vi "Motion_one_way_ver2_lin_sin.vi"(7 "Parameters":T1={"T"=2000.0, "Linear or sine?"=0.0, "Buffer size"=0.5, "Buffer power"=3.0}, 8 "Error IN":errorcluster, 9 "previousSTATE":dbl[][](array[numeric]), 10 "nextSTATE":dbl[][](array[numeric]), 11 "Constants IN":T3) -> (0 "Error OUT":errorcluster, 2 "Motion Sequence":T2, 3 "Constants OUT":T3)   [LabVIEW 2019]
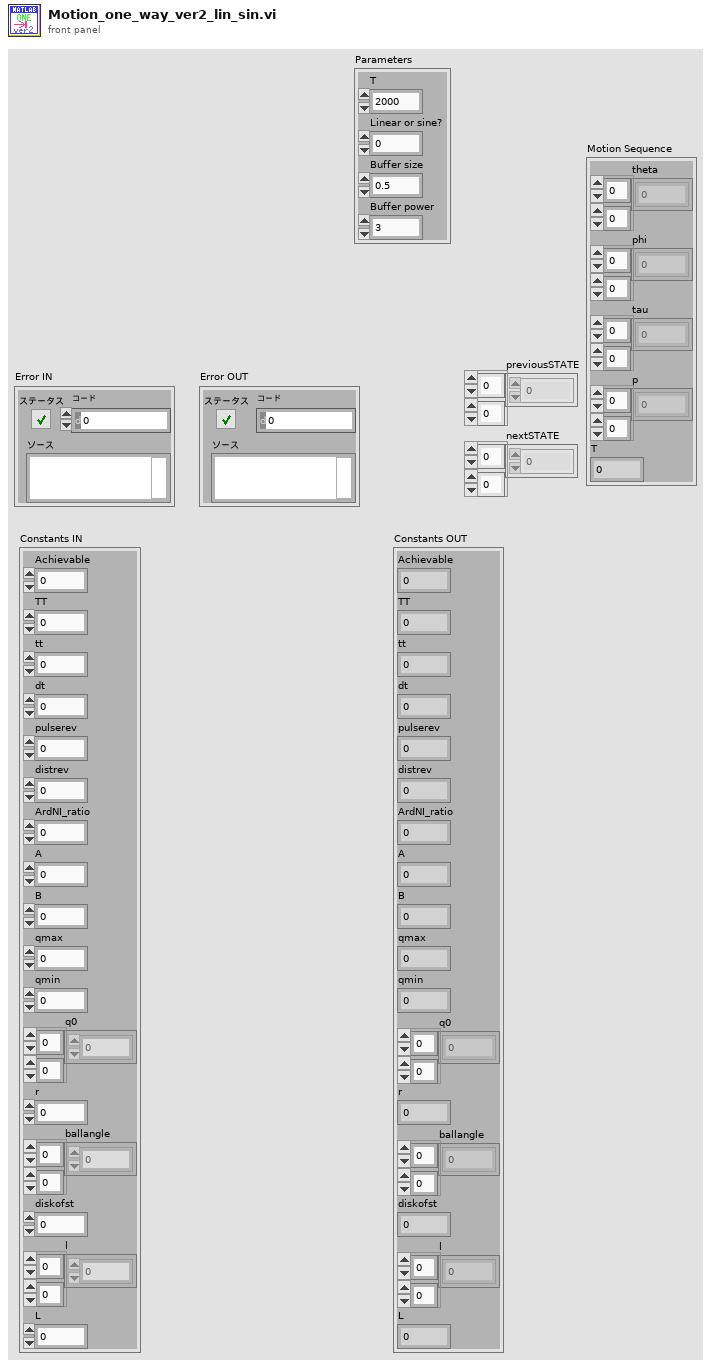
[diagram p1: front panel]
types:
  T1 = cluster{"T":dbl, "Linear or sine?":dbl, "Buffer size":dbl, "Buffer power":dbl}
  T2 = cluster{"theta":dbl[][], "phi":dbl[][], "tau":dbl[][], "p":dbl[][], "T":dbl}
  T3 = cluster{"Achievable":dbl, "TT":dbl, "tt":dbl, "dt":dbl, "pulserev":dbl, "distrev":dbl, "ArdNI_ratio":dbl, "A":dbl, "B":dbl, "qmax":dbl, "qmin":dbl, "q0":dbl[][], "r":dbl, "ballangle":dbl[][], "diskofst":dbl, "l":dbl[][], "L":dbl}
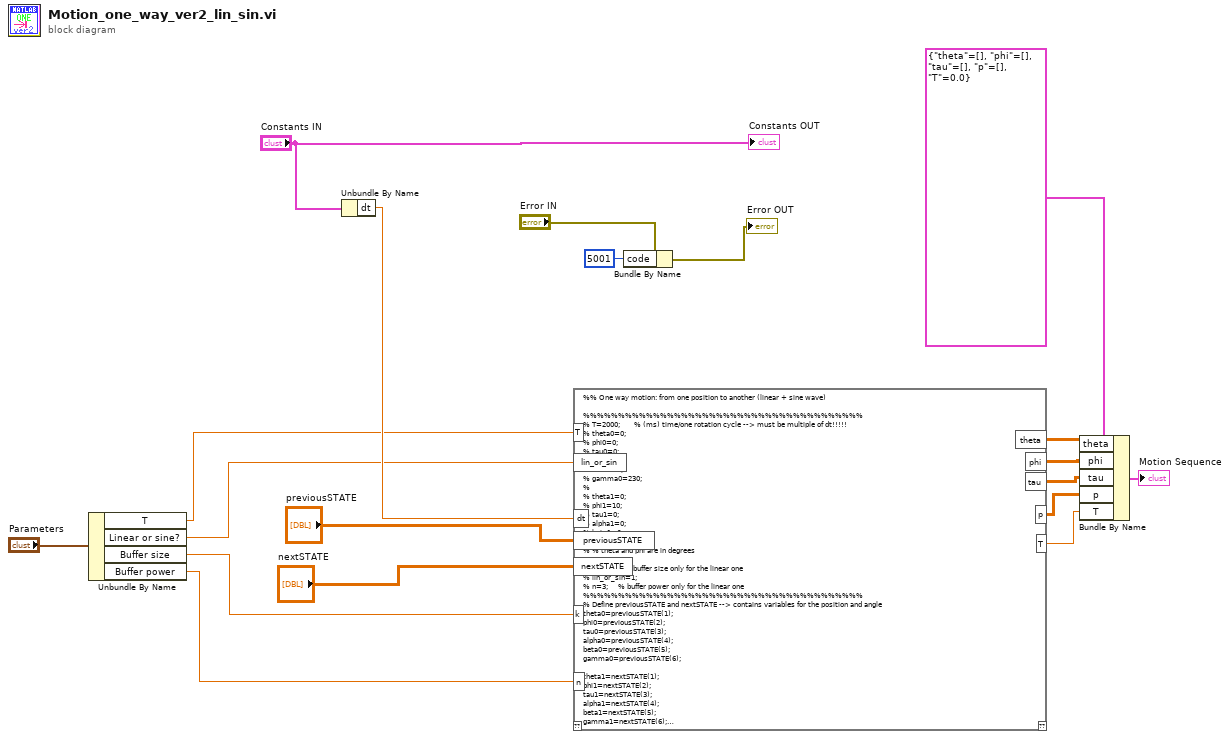
[diagram p0: block diagram]
diagram:
  n1 = Unbundle By Name("Parameters") -> ("T"=w4:dbl, "Linear or sine?"=w3:dbl, "Buffer size"=w2:dbl, "Buffer power"=w1:dbl)
  n2 = Unbundle By Name("Constants IN") -> ("dt"=w6:dbl)
  n3 = script code="%% One way motion: from one position to another (linear + sine wave)\n\n%%%%%%%%%%%%%%%%%%%%%%%%%%%%%%%%%%%%%%%%\n% T=2000;\t\t\t\t\t\t\t% (ms) time/one rotation cycle --> must be multiple of dt!!!!!\n% theta0=0;\n% phi0=0;\n% tau0=0;\n% alpha0=0;\n% beta0=0;\n% gamma0=230;\n% \n% theta1=0;\n% phi1=10;\n% tau1=0;\n% alpha1=0;\n% beta1=0;\n% gamma1=230;\n% % theta and phi are in degrees\n% \n% k=0.5;\t\t\t\t\t% buffer size only for the linear one \n% lin_or_sin=1;\n% n=3;\t\t\t\t\t% buffer power only for the linear one\n%%%%%%%%%%%%%%%%%%%%%%%%%%%%%%%%%%%%%%%%\n% Define previousSTATE and nextSTATE --> contains variables for the position and angle\ntheta0=previousSTATE(1);\nphi0=previousSTATE(2);\ntau0=previousSTATE(3);\nalpha0=previousSTATE(4);\nbeta0=previousSTATE(5);\ngamma0=previousSTATE(6);\n\ntheta1=nextSTATE(1);\nphi1=nextSTATE(2);\ntau1=nextSTATE(3);\nalpha1=nextSTATE(4);\nbeta1=nextSTATE(5);\ngamma1=nextSTATE(6);\nlin_or_sin;\n%%%%%%%%%%%%%%%%%%%%%%%%%%%%%%%%%%%%%%%%\n\n\ntheta0=(pi/180)*theta0;\nphi0=(pi/180)*phi0;\ntau0=(pi/180)*tau0;\ntheta1=(pi/180)*theta1;\nphi1=(pi/180)*phi1;\ntau1=(pi/180)*tau1;\n\nif k>0.5\n\tk=0.5;\nend\n\ntheta=zeros(1,1,T/dt+1);\nphi=zeros(1,1,T/dt+1);\ntau=zeros(1,1,T/dt+1);\np=zeros(3,6,T/dt+1);\nif k<=dt/T\n\tif theta0==theta1\n\t\ttheta=zeros(1,1,T/dt+1)+theta0;\n\telse\n\t\ttheta(1,1,:)=[theta0:(theta1-theta0)*dt/T:theta1];\n\tend\n\tif phi0==phi1\n\t\tphi=zeros(1,1,T/dt+1)+phi0;\n\telse\n\t\tphi(1,1,:)=[phi0:(phi1-phi0)*dt/T:phi1];\n\tend\n\tif tau0==tau1\n\t\ttau=zeros(1,1,T/dt+1)+tau0;\n\telse\n\t\ttau(1,1,:)=[tau0:(tau1-tau0)*dt/T:tau1];\n\tend\n\t\n\tp0=alpha0;\n\tp1=alpha1;\n\tdimension=1;\n\tif p0==p1\n\t\tprep=zeros(1,6,T/dt+1)+p0;\n\t\tp(dimension,:,:)=prep;\n\telse\n\t\tprep=zeros(1,1,T/dt+1);\n\t\tprep(1,1,:)=[p0:(p1-p0)*dt/T:p1];\n\t\tprep=zeros(1,6,T/dt+1)+prep;\n\t\tp(dimension,:,:)=prep;\n\tend\n\t\n\tp0=beta0;\n\tp1=beta1;\n\tdimension=2;\n\tif p0==p1\n\t\tprep=zeros(1,6,T/dt+1)+p0;\n\t\tp(dimension,:,:)=prep;\n\telse\n\t\tprep=zeros(1,1,T/dt+1);\n\t\tprep(1,1,:)=[p0:(p1-p0)*dt/T:p1];\n\t\tprep=zeros(1,6,T/dt+1)+prep;\n\t\tp(dimension,:,:)=prep;\n\tend\n\t\n\tp0=gamma0;\n\tp1=gamma1;\n\tdimension=3;\n\tif p0==p1\n\t\tprep=zeros(1,6,T/dt+1)+p0;\n\t\tp(dimension,:,:)=prep;\n\telse\n\t\tprep=zeros(1,1,T/dt+1);\n\t\tprep(1,1,:)=[p0:(p1-p0)*dt/T:p1];\n\t\tprep=zeros(1,6,T/dt+1)+prep;\n\t\tp(dimension,:,:)=prep;\n\tend\nelse\n\tx0=[0:dt/T:1];\n\tif lin_or_sin~=1\n\t\ta0=1/(k^(n-1)*(2*k+n*(1-2*k)));\n\t\tx0=[0:dt/T:1];\n\t\tprey1=a0*x0.^n;\n\t\tprey1(x0>=k)=0;\n\t\tprey2=a0*k^n+n*a0*k^(n-1)*(x0-k);\n\t\tprey2(x0<k | x0>=1-k)=0;\n\t\tprey3=1-a0*(1-x0).^n;\n\t\tprey3(x0<1-k)=0;\n\t\tprey=prey1+prey2+prey3;\n\telse\n\t\tprey=(1/2)*(1-cos(pi*x0));\n\tend\n\tL0=theta0;\n\tL1=theta1;\n\ty=(L1-L0).*prey+L0;\n\ttheta(1,1,:)=y;\n\t\n\tL0=phi0;\n\tL1=phi1;\n\ty=(L1-L0).*prey+L0;\n\tphi(1,1,:)=y;\n\t\n\tL0=tau0;\n\tL1=tau1;\n\ty=(L1-L0).*prey+L0;\n\ttau(1,1,:)=y;\n\t\n\tL0=alpha0;\n\tL1=alpha1;\n\tprep=zeros(1,1,T/dt+1);\n\ty=(L1-L0).*prey+L0;\n\tprep(1,1,:)=y;\n\tprep=zeros(1,6,T/dt+1)+prep;\n\tp(1,:,:)=prep;\n\t\n\tL0=beta0;\n\tL1=beta1;\n\tprep=zeros(1,1,T/dt+1);\n\ty=(L1-L0).*prey+L0;\n\tprep(1,1,:)=y;\n\tprep=zeros(1,6,T/dt+1)+prep;\n\tp(2,:,:)=prep;\n\t\n\tL0=gamma0;\n\tL1=gamma1;\n\tprep=zeros(1,1,T/dt+1);\n\ty=(L1-L0).*prey+L0;\n\tprep(1,1,:)=y;\n\tprep=zeros(1,6,T/dt+1)+prep;\n\tp(3,:,:)=prep;\nend"("previousSTATE"="previousSTATE", "nextSTATE"="nextSTATE", "T"=w4, "dt"=w6, "k"=w2, "lin_or_sin"=w3, "n"=w1) -> ("theta"=w16:dbl[][], "phi"=w15:dbl[][], "tau"=w14:dbl[][], "p"=w13:dbl[][], "T"=w9:dbl)  [unwired: 1 in, 1 out]
  n4 = Bundle By Name(cluster="Error IN", "code"=5001) -> (→"Error OUT":errorcluster)
  n5 = Bundle By Name(cluster=T2 {"theta"=[], "phi"=[], "tau"=[], "p"=[], "T"=0.0}, "theta"=w16, "phi"=w15, "tau"=w14, "p"=w13, "T"=w9) -> (→"Motion Sequence":T2)
  "Constants OUT" <- "Constants IN"
